vi "Host_Edge.vi"(9 "Prev":bool, 10 "Timed Out":bool, 11 "Status":u16) -> (1 "Next":bool, 2 "Falling":bool, 3 "Rising":bool)   [LabVIEW 2018]
doc: "Use this template to build a VI to use as a subVI."
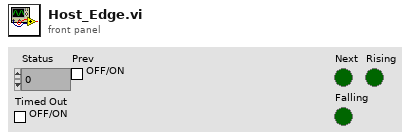
[diagram p1: front panel]
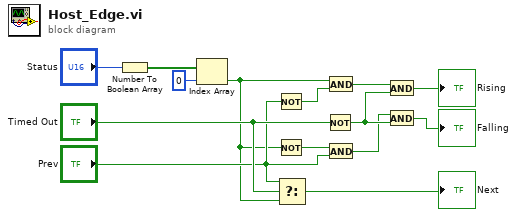
[diagram p0: block diagram]
diagram:
  n1 = Number To Boolean Array(number="Status") -> (Boolean array=w13:bool[])
  n2 = Index Array(array=w13, index=0) -> (element=w9:bool)
  n3 = Not(x="Prev") -> (.not. x?=w7:bool)
  n4 = Not(x=w9) -> (.not. x?=w4:bool)
  n5 = Select(t="Prev", s="Timed Out", f=w9) -> (s? t:f=→"Next":bool)
  n6 = Not(x="Timed Out") -> (.not. x?=w5:bool)
  n7 = And(x=w9, y=w7) -> (x .and. y?=w6:bool)
  n8 = And(x=w4, y="Prev") -> (x .and. y?=w3:bool)
  n9 = And(x=w6, y=w5) -> (x .and. y?=→"Rising":bool)
  n10 = And(x=w3, y=w5) -> (x .and. y?=→"Falling":bool)
